vi "Parse Set Marker.vi"(8 "error in (no error)":errorcluster caption="에러 입력(에러 없음)", 10 "JSON string":string, 11 "Instrument Manager 입력":refnum<class "Instrument Manager.lvclass">) -> (0 "error out":errorcluster caption="에러 출력", 1 "Marker Index":i32, 2 "Set Marker Param":T1, 3 "Instrument Manager 출력":refnum<class "Instrument Manager.lvclass">)   [LabVIEW 2023, in "Instrument Manager.lvclass"]
uses:
  Instrument Manager.lvclass
  Param Definition/Set Marker Param.ctl
  Instrument Manager.lvclass/Instrument Manager.ctl
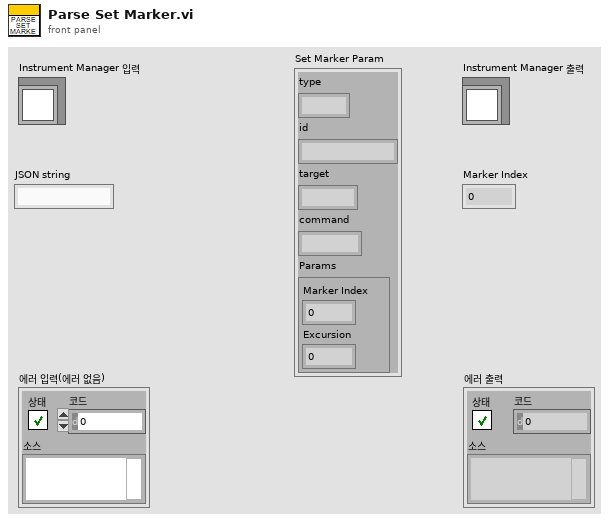
[diagram p1: front panel]
types:
  T1 = typedef "Instrument Manager.lvclass/Set Marker Param.ctl" = cluster{"type":string, "id":string, "target":string, "command":string, "Params":cluster{"Marker Index":i32, "Excursion":dbl}}
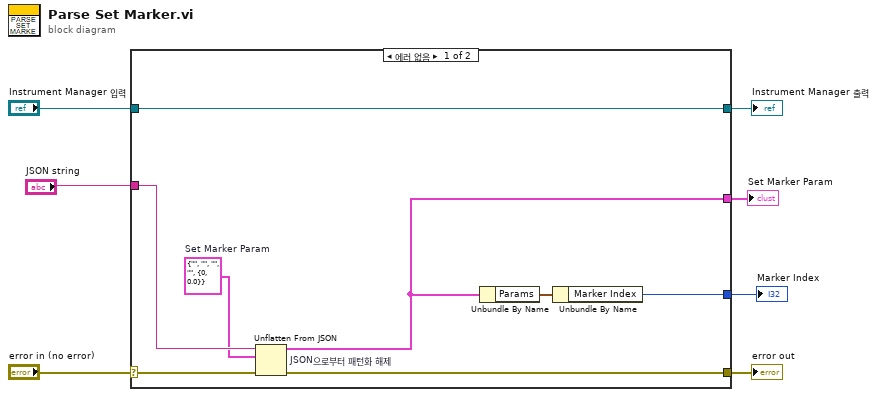
[diagram p0: block diagram]
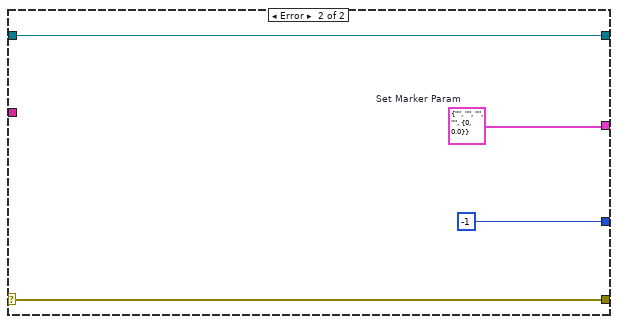
[diagram p2: hidden frame]
diagram:
  n1 = case shown="에러 없음" "error in (no error)" {
    selector: "error in (no error)" -> [w13 w19]
    tunnel: [w12 w19] -> w6
    tunnel: [w15 w18] -> w4
    tunnel: "Instrument Manager 입력" -> [w15 w18]
    tunnel: "JSON string" -> [w14 _]
    tunnel: [w9 w17] -> w2
    tunnel: [w8 -1 ("Marker Index")] -> w1
    frame No Error {
      w11 = T1 {"type"="", "id"="", "target"="", "command"="", "Params"={"Marker Index"=0, "Excursion"=0.0}}  # Set Marker Param
      n2 = Unflatten From JSON "JSON으로부터 패턴화 해제"(JSON string=w14, type and defaults=w11, error in (no error)=w13) -> (value=w9:T1, error out=w12:errorcluster)  [unwired: 4 in]
      n3 = Unbundle By Name(w9) -> ("Params"=w10:cluster{"Marker Index":i32, "Excursion":dbl})
      n4 = Unbundle By Name(w10) -> ("Marker Index"=w8:i32)
    }
    frame Error {
      w17 = T1 {"type"="", "id"="", "target"="", "command"="", "Params"={"Marker Index"=0, "Excursion"=0.0}}  # Set Marker Param
    }
  }
  "error out" <- w6
  "Instrument Manager 출력" <- w4
  "Set Marker Param" <- w2
  "Marker Index" <- w1
